vi "RT_lab7.vi"() -> ()   [LabVIEW 2025]
uses:
  <vilib>/dex/Flush And Wait Empty Condition.ctl
  RT_Cmd.ctl
  Command.ctl
  vi/thresholds.ctl
  <vilib>/Utility/error.llb/Error Cluster From Error Code.vi
  <vilib>/rvi/errors/niLvFpgaAdjustHostInterfaceError.vi
  <vilib>/FPGAPlugInAG/Dynamic/niLvFpga_Close_Dynamic.vi
  <vilib>/rvi/interface/nirviReadWriteControl/nirviReadWriteControl.xnode
  <vilib>/rvi/interface/nirviMethod/nirviMethod.xnode
  <vilib>/rvi/interface/nirviCloseFPGA/nirviCloseFPGA.xnode
  NiFpgaLv.dll
  <vilib>/rvi/interface/Simulation/niFpgaSimulationCallBeginRW.vi
  <vilib>/FPGAPlugInAG/Dynamic/niLvFpga_ReadFifo_Dynamic.vi
  <vilib>/rvi/errors/niLvFpgaMergeErrorWithErrorCode.vi
panel:
  out "Elements Remaining":u32
  out "Waveform Graph":i16[][](graph)
  out "error out":errorcluster
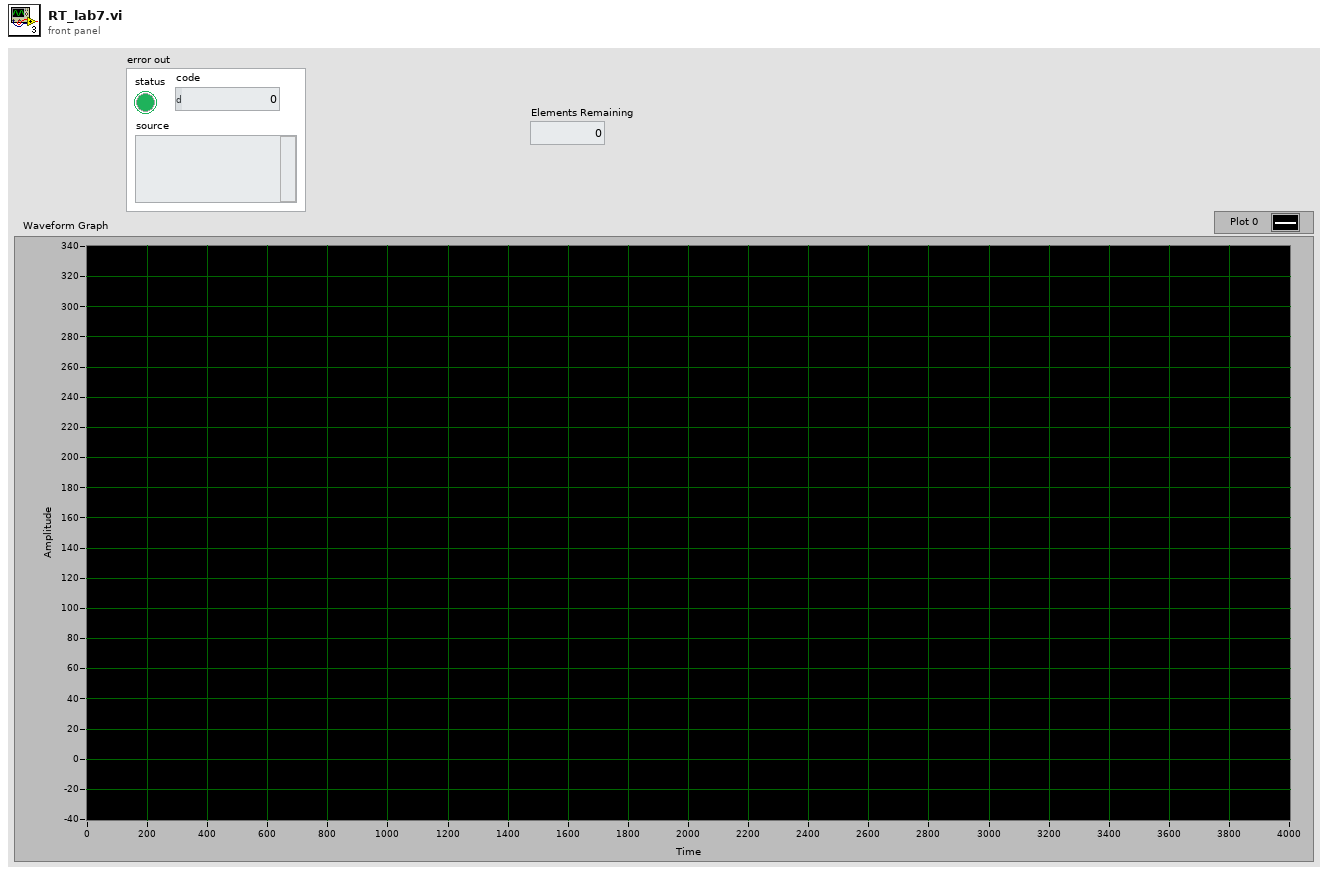
[diagram p1: front panel]
types:
  T1 = typedef "Flush And Wait Empty Condition.ctl" = u8
  T2 = typedef "RT_Cmd.ctl" = cluster{"command":T3, "parameters":T4}
  T3 = typedef "Command.ctl" = enum16{"threshold_config", "manual_trigger", "stop"}
  T4 = typedef "thresholds.ctl" = cluster{"Thr_X":i16, "Thr_Y":i16, "Thr_Z":i16}
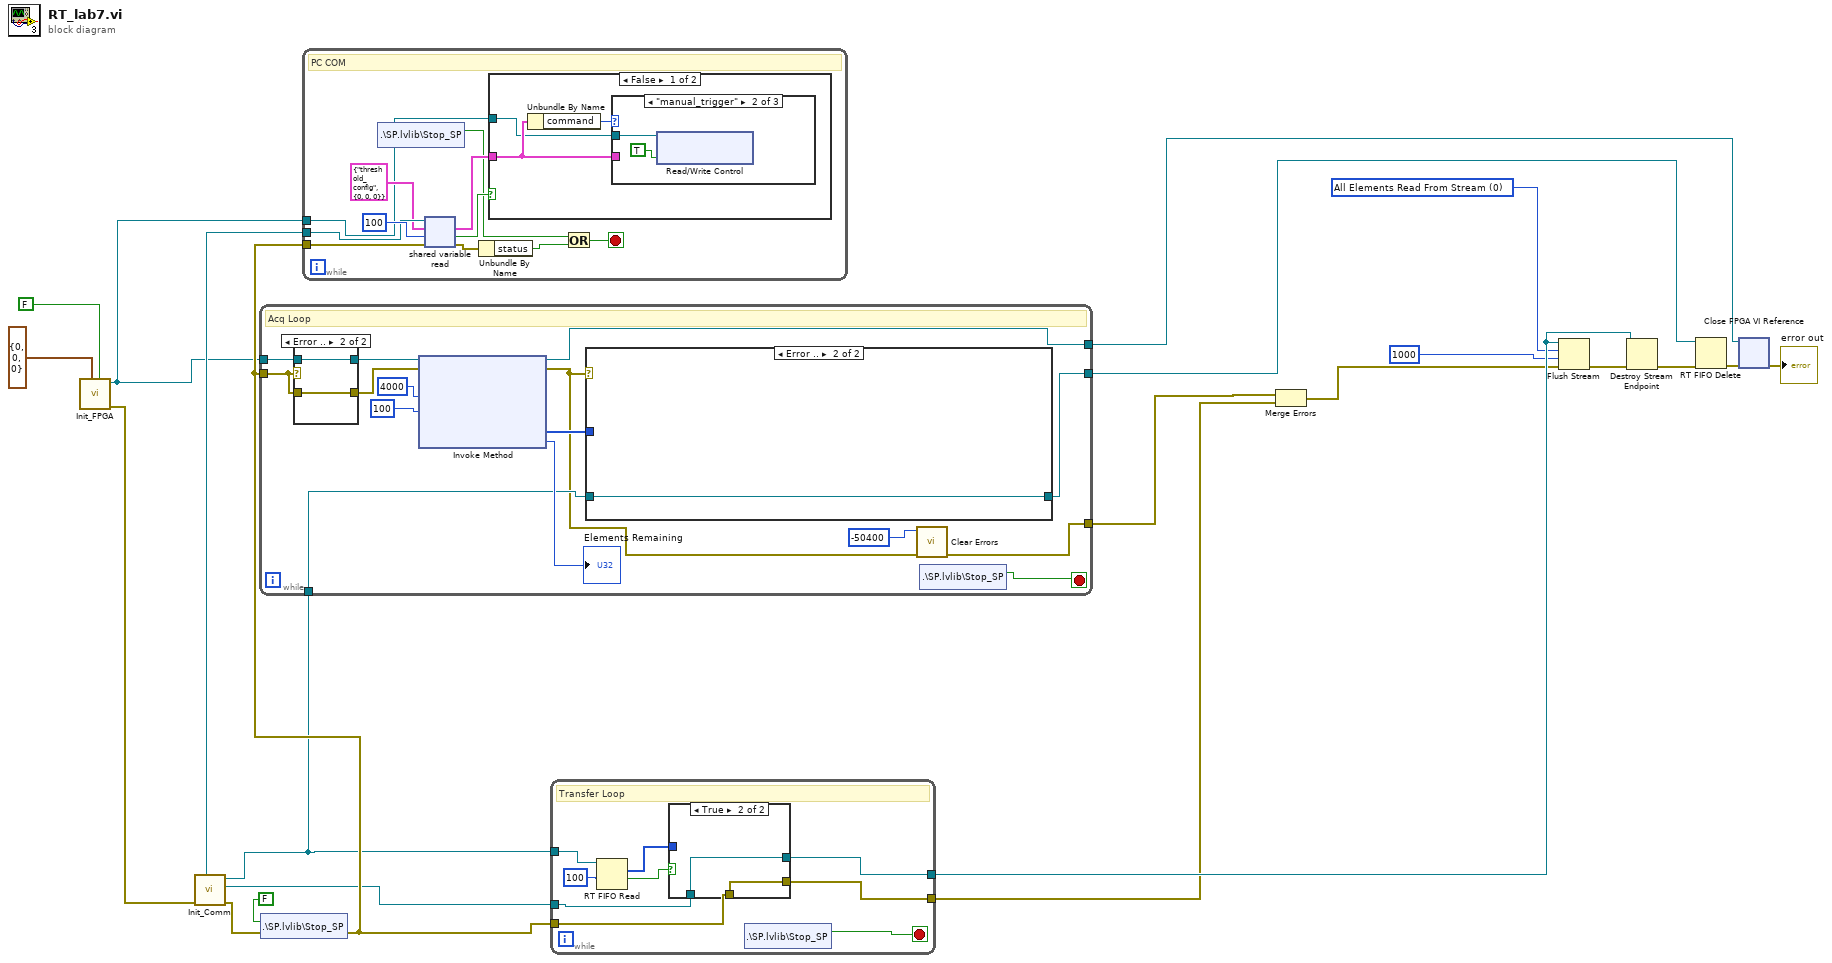
[diagram p0: block diagram]
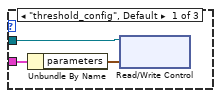
[diagram p2: hidden frame]
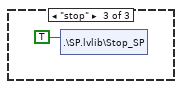
[diagram p3: hidden frame]
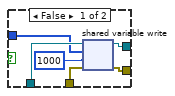
[diagram p5: hidden frame]
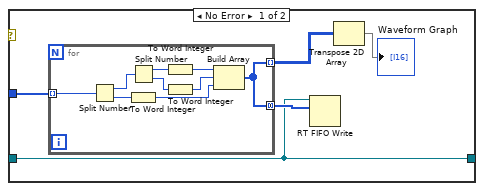
[diagram p6: hidden frame]
diagram:
  w19 = T1 0 items=["All Elements Read From Stream", "All Elements Available for Reading"] ("wait condition")
  n1 = call "Init_FPGA.vi"("manual trigger"=FALSE, "Threshold"=cluster{"Thr_X":i16, "Thr_Y":i16, "Thr_Z":i16} {"Thr_X"=0, "Thr_Y"=0, "Thr_Z"=0}) -> ("error out"=w16:errorcluster, "FPGA VI Reference Out"=w1:refnum<k20>)  [unwired: 8 in]
  n2 = call "Init_Comm.vi"("error in"=w16) -> ("error out"=w9:errorcluster, "writer endpoint ref out"=w5:refnum<k21>, "rt fifo ref out"=w6:refnum<k33>, "reader endpoint ref out"=w4:refnum<k21>)  [unwired: 7 in]
  n3 = shared-variable ".\\SP.lvlib\\Stop_SP"(FALSE ("Stop_SP"), error in=w9) -> (error out=w7:errorcluster)
  n4 = while {
    tunnel: w1 -> [w33]
    tunnel: w7 -> [w32]
    tunnel: [w31] -> w11
    tunnel: [w26] -> w14
    tunnel: w6 -> [w28]
    tunnel: [w24] -> w10
    stop <- w23 stop-if-true
    # "Acq Loop"
    n5 = case shown="Error .." w32 {
      tunnel: w33 -> [w54 w56]
      tunnel: [w54 w56] -> w37
      tunnel: w32 -> [w53 w55]
      tunnel: [w53 w55] -> w36
      frame No Error {
      }
      frame Error {
      }
    }
    n6 = xnode "Invoke Method"("FPGA VI Reference In"=w37, "error in"=w36, "Number of Elements"=u32 4000, "Timeout (ms)"=100) -> ("FPGA VI Reference Out"=w31:refnum<k20>, "error out"=w27:errorcluster, "Data"=w30:u64[], "Elements Remaining"=→"Elements Remaining":u32)
    n7 = case shown="Error .." w27 {
      tunnel: w30 -> [w42 _]
      tunnel: w28 -> [w38 w52]
      tunnel: [w38 w52] -> w24
      frame No Error {
        n8 = for {
          tunnel: w42 -> [w51] mode=indexing
          tunnel: [w43] -> w40 mode=concatenating
          tunnel: [w43] -> w39 mode=indexing
          n9 = Split Number(x=w51) -> (hi(x)=w50:u32, lo(x)=w47:u32)
          n10 = To Word Integer(number=w47) -> (16bit integer=w44:i16)
          n11 = Split Number(x=w50) -> (hi(x)=w49:u16, lo(x)=w48:u16)
          n12 = To Word Integer(number=w49) -> (16bit integer=w46:i16)
          n13 = To Word Integer(number=w48) -> (16bit integer=w45:i16)
          n14 = Build Array(w46, w45, w44) -> (w43:i16[])
        }
        n15 = RT FIFO Write(0:w38, 1:w40) -> ()  [unwired: 3 in, 4 out]
        n16 = Transpose 2D Array(2D array=w39) -> (transposed array=→"Waveform Graph":i16[][])
      }
      frame Error {
      }
    }
    n17 = call <vilib>:"Clear Errors.vi"("error in (no error)"=w27, "specific error code to clear (0: all)"=-50400) -> ("error out"=w26:errorcluster)  [unwired: 4 in, 1 out]
    n18 = shared-variable ".\\SP.lvlib\\Stop_SP"() -> (w23:bool)  [unwired: 1 in, 1 out]
  }
  n19 = while {
    tunnel: w7 -> [w67]
    tunnel: w4 -> [w65]
    tunnel: w1 -> [w59]
    stop <- w60 stop-if-true
    # "PC COM"
    n20 = shared-variable ".\\SP.lvlib\\Stop_SP"() -> (w61:bool)  [unwired: 1 in, 1 out]
    n21 = shared-variable-read(w65, w67, T2 {"command"=enum."threshold_config", "parameters"={"Thr_X"=0, "Thr_Y"=0, "Thr_Z"=0}} ("data"), 100 ("timeout ms (-1)")) -> (w58:errorcluster, w63:bool, w62:T2)  [unwired: 1 out]
    n22 = Unbundle By Name(w58) -> ("status"=w57:bool)
    n23 = case shown="False" w63 {
      tunnel: w62 -> [w69 _]
      tunnel: w59 -> [w68 _]
      frame False {
        n24 = Unbundle By Name(w69) -> ("command"=w70:T3)
        n25 = case shown="\"manual_trigger\"" w70 {
          tunnel: w69 -> [w73 _ _]
          tunnel: w68 -> [w72 w75 _]
          frame "threshold_config", Default {
            n26 = Unbundle By Name(w73) -> ("parameters"=w71:T4)
            n27 = xnode "Read/Write Control"("FPGA VI Reference In"=w72, "Threshold"=w71) -> ()  [unwired: 1 in, 2 out]
          }
          frame "manual_trigger" {
            n28 = xnode "Read/Write Control"("FPGA VI Reference In"=w75, "manual trigger"=TRUE) -> ()  [unwired: 1 in, 2 out]
          }
          frame "stop" {
            n29 = shared-variable ".\\SP.lvlib\\Stop_SP"(TRUE ("Stop_SP")) -> ()  [unwired: 1 in, 1 out]
          }
        }
      }
      frame True {
      }
    }
    n30 = Or(x=w61, y=w57) -> (x .or. y?=w60:bool)
  }
  n31 = while {
    tunnel: w6 -> [w85]
    tunnel: w5 -> [w82]
    tunnel: [w80] -> w21
    tunnel: [w79] -> w15
    tunnel: w7 -> [w81]
    stop <- w77 stop-if-true
    # "Transfer Loop"
    n32 = RT FIFO Read(0:w85, 2:100 ("timeout in ms (0)")) -> (9:w78:i16[], 10:w83:bool)  [unwired: 2 in, 3 out]
    n33 = case shown="True" w83 {
      tunnel: w82 -> [w91 w92]
      tunnel: w81 -> [w90 w93]
      tunnel: [w89 w92] -> w80
      tunnel: [w88 w93] -> w79
      tunnel: w78 -> [w86 _]
      frame False {
        n34 = shared-variable-write(w91, w90, w86, 1000 ("timeout ms (-1)")) -> (w89:refnum<k21>, w88:errorcluster)  [unwired: 1 out]
      }
      frame True {
      }
    }
    n35 = shared-variable ".\\SP.lvlib\\Stop_SP"() -> (w77:bool)  [unwired: 1 in, 1 out]
  }
  n36 = Merge Errors(w14, w15) -> (w13:errorcluster)
  n37 = Flush Stream(8:w13, 9:1000 ("timeout in ms (-1)"), 10:w19, 11:w21) -> (0:w20:errorcluster)  [unwired: 2 out]
  n38 = Destroy Stream Endpoint(8:w20, 11:w21) -> (0:w18:errorcluster)
  n39 = RT FIFO Delete(0:w10, 3:w18) -> (11:w17:errorcluster)  [unwired: 1 in]
  n40 = xnode "Close FPGA VI Reference"("FPGA VI Reference In"=w11, "error in"=w17) -> ("error out"=→"error out":errorcluster)
